vi "Supervisor_Loop.vi"(8 "error in (no error)":errorcluster={"status"=FALSE, "code"=0, "source"="\"\""}, 10 "RunContext":string="STATE_READY", 11 "Supervisor message queue":string="MSG_START") -> (0 "error out":errorcluster={"status"=FALSE, "code"=0, "source"="\"\""}, 2 "status ok":bool, 3 "State transitions/events":string)   [LabVIEW 2026]
doc: "INTENT: Supervisory Message Handling Loop dequeuing runtime messages and transitioning engine states."
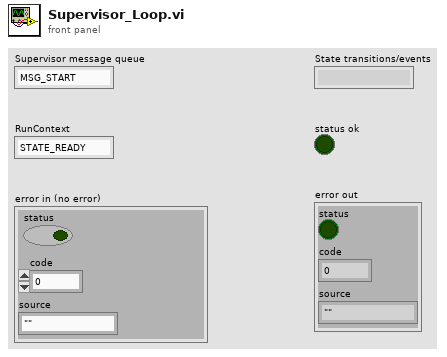
[diagram p1: front panel]
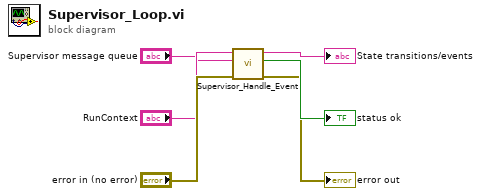
[diagram p0: block diagram]
diagram:
  n1 = call "Supervisor_Handle_Event.vi"("error in (no error)"="error in (no error)", "RuntimeMessage"="Supervisor message queue", "Current run state"="RunContext") -> ("error out"=→"error out":errorcluster, "status ok"=→"status ok":bool, "Updated state and effects"=→"State transitions/events":string)  [unwired: 6 in]
